vi "Get Device Settings.vi"(8 "error in (no error)":errorcluster, 11 "Device Session Name":string) -> (0 "error out":errorcluster, 3 "Device Settings":T1)   [LabVIEW 2021]
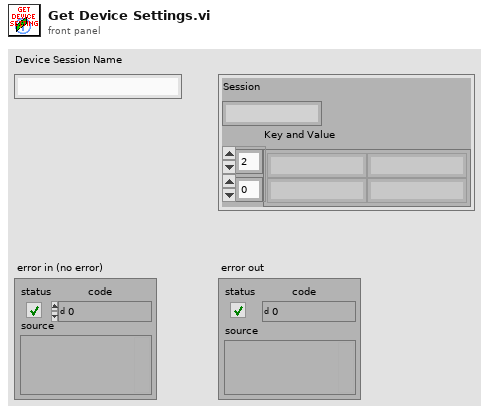
[diagram p1: front panel]
types:
  T1 = cluster{"Session":string, "Key and Value":string[][]}
  T2 = typedef "Device Settings.ctl" = cluster{"Session":string, "Key and Value":string[][]}
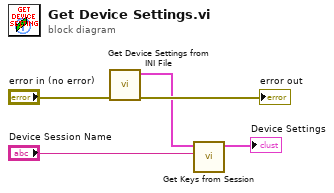
[diagram p0: block diagram]
diagram:
  n1 = call "Get Device Settings from INI File.vi"("error in (no error)"="error in (no error)") -> ("error out"=→"error out":errorcluster, "Device Settings"=w1:T2[])  [unwired: 9 in]
  n2 = call "Get Keys from Session .vi"("Session Name"="Device Session Name", "Device Settings"=w1) -> ("Cluster"=→"Device Settings":T1)  [unwired: 9 in]
